vi "waveform_chart.vi"() -> ()   [LabVIEW 2018]
panel:
  in  "stop":bool
  out "Waveform Graph":dbl[](graph)
  out "Waveform Chart":dbl(graph)
  # "chart has history that allows it to keep prior data"
  # "graph dosen't have memory"
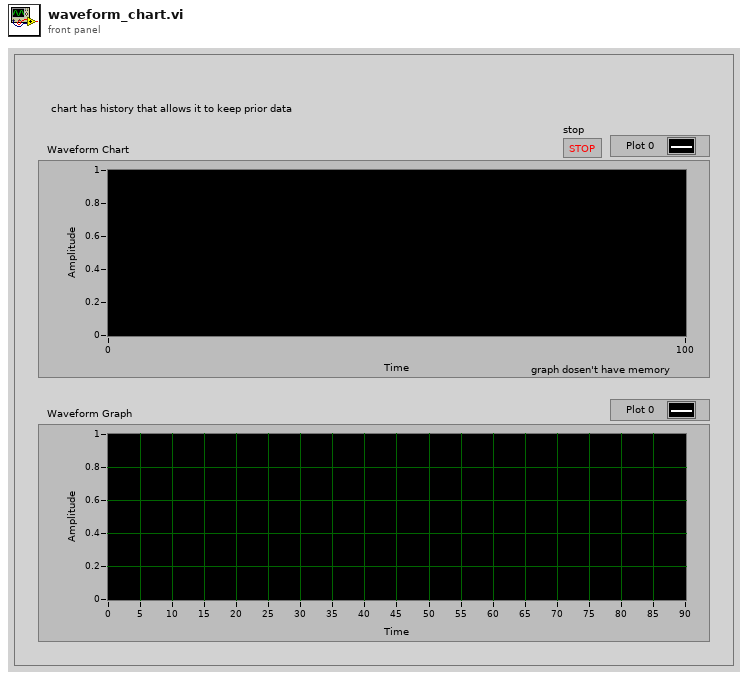
[diagram p1: front panel]
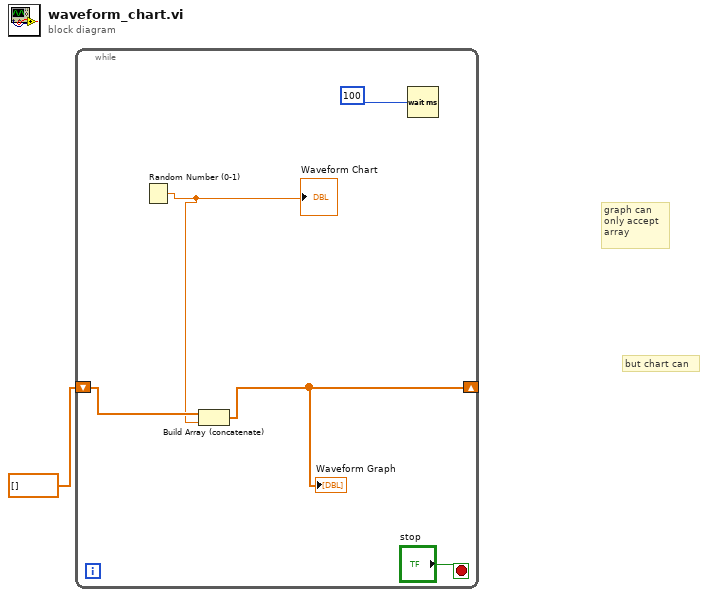
[diagram p0: block diagram]
diagram:
  # "but chart can"
  # "graph can \nonly accept \narray"
  n1 = while {
    shift-right: [w2] -> _
    shift-left: dbl[] [] ("Waveform Graph") -> [w4]
    stop <- "stop" stop-if-true
    n2 = Random Number (0-1)() -> (number: 0 to 1=w3:dbl)
    "Waveform Chart" <- w3
    n3 = Build Array (concatenate)(w4, w3) -> (w2:dbl[])
    "Waveform Graph" <- w2
    n4 = Wait (ms)(milliseconds to wait=100) -> ()  [unwired: 1 out]
  }
